vi "test Import Configuration File (Sequential Use).vi"(8 "error in":errorcluster, 11 "TestCase in":refnum<class "Import.lvclass">) -> (0 "error out":errorcluster, 3 "TestCase out":refnum<class "Import.lvclass">)   [LabVIEW 2020, in "Import.lvclass"]
uses:
  Import.lvclass
  Import.lvclass/Import.ctl
  C:/Program Files/National Instruments/LabVIEW 2026/vi.lib/addons/_JKI Toolkits/VI Tester/TestCase.llb/TestCase.lvclass
  <vilib>/addons/_JKI Toolkits/VI Tester/TestCase.llb/TestCase.lvclass
  Import/ARINC 429 Import.lvlib
  <userlib>/_OpenG.lib/appcontrol/appcontrol.llb/openg_application_control.lvlib
  <vilib>/NI/VeriStand Custom Device Testing Tools/VeriStandTestUtilities/VeriStandTestUtilities.lvlib
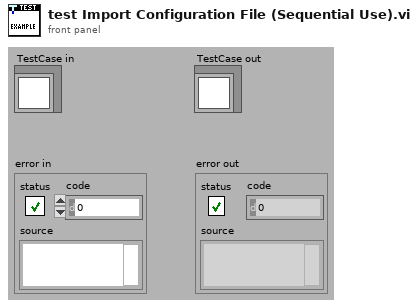
[diagram p1: front panel]
types:
  T1 = typedef "VS Channels Definition for All Labels on Hardware Channel.ctl" = cluster{"hardware channel":i32, "direction":T2, "labels":T3[], "speed":T8}
  T2 = typedef "Direction.ctl" = enum16{"Rx", "Tx"}
  T3 = typedef "VS Channels Definition for Label.ctl" = cluster{"label (Dec)":u32, "parameters":T4[], "SDI value":u8, "SDI enabled":bool, "transfer type":T7, "create timestamp":bool, "transmit period":u32}
  T4 = typedef "VS Channel Definition for Parameter.ctl" = cluster{"name":string, "unit":string, "Parameter":T5}
  T5 = typedef "Parameter Definition.ctl" = cluster{"start index":i32, "size":i32, "encoding":T6, "signed":bool, "scale multiplier":dbl, "scale offset":dbl, "default value":dbl}
  T6 = typedef "Encoding and Decoding.lvlib/Encoding.ctl" = enum16{"BNR", "BCD", "Discrete"}
  T7 = typedef "Transfer Type.ctl" = enum16{"Scheduled", "Acyclic", "Block", "Strobe"}
  T8 = typedef "Transfer Speed.ctl" = enum16{"LO (12.5 kb/s)", "HI (100 kb/s)"}
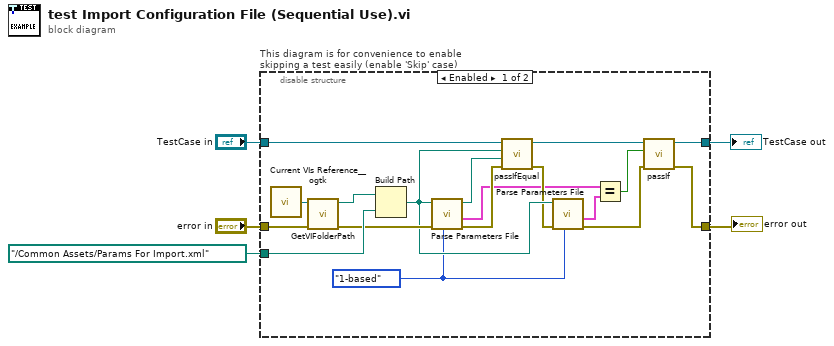
[diagram p0: block diagram]
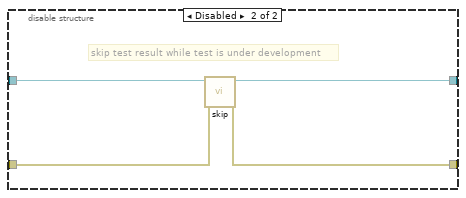
[diagram p2: hidden frame]
diagram:
  n1 = disable-structure "This diagram is for convenience to enable skipping a test easily (enable 'Skip' case)" shown="Enabled" {
    disable-tunnel: "TestCase in" -> [w23 w27]
    disable-tunnel: [w17 w25] -> w2
    disable-tunnel: [w18 w26] -> w4
    disable-tunnel: "error in" -> [w21 w24]
    disable-tunnel: path "../Common Assets/Params For Import.xml" ("Absolute or Relative Path") -> [w20 _]
    frame Enabled {
      w6 = enum16{"0-based", "1-based"}."1-based" ("ch indexing (0-based)")
      n2 = call <userlib>:"Current VIs Reference__ogtk.vi"() -> ("Current VI's reference"=w22:refnum<vi>)  [unwired: 5 in]
      n3 = call <vilib>:"GetVIFolderPath.vi"("error in (no error)"=w21, "VI Reference in"=w22) -> ("error out"=w19:errorcluster, "VI Folder Path out"=w14:path)  [unwired: 8 in]
      n4 = Build Path(base path=w14, name or relative path=w20) -> (appended path=w15:path)
      n5 = call "Parse Parameters File.vi"("ch indexing (0-based)"=w6, "error in"=w19, "path to XML document"=w15) -> ("error out"=w13:errorcluster, "ports"=w8:T1[], "path to XML document out"=w9:path)  [unwired: 6 in]
      n6 = call-dynamic "passIfEqual.vi"("error in (no error)"=w13, "y"=w9, "x"=w15, "TestCase in"=w23) -> ("error out"=w11:errorcluster, "TestCase out"=w12:refnum<class "Import.lvclass">)  [unwired: 6 in]
      n7 = call "Parse Parameters File.vi"("ch indexing (0-based)"=w6, "error in"=w11, "path to XML document"=w15) -> ("error out"=w10:errorcluster, "ports"=w7:T1[])  [unwired: 6 in, 1 out]
      n8 = Equal?(x=w8, y=w7) -> (x = y?=w16:bool)
      n9 = call-dynamic "passIf.vi"("error in (no error)"=w10, "pass"=w16, "TestCase in"=w12) -> ("error out"=w18:errorcluster, "TestCase out"=w17:refnum<class "Import.lvclass">)  [unwired: 7 in]
    }
    frame Disabled {
      # "skip test result while test is under development"
      n10 = call <vilib>:"skip.vi"("error in (no error)"=w24, "TestCase in"=w27) -> ("error out"=w26:errorcluster, "TestCase out"=w25:refnum<class "Import.lvclass">)  [unwired: 8 in]
    }
  }
  "error out" <- w4
  "TestCase out" <- w2
